vi "ShowErrorAndStatusAndStop.vi"(8 "error in":errorcluster, 10 "measured value in":dbl, 11 "measurement setting in":T1) -> ()   [LabVIEW 2011]
doc: "Shows errors and status of measurement."
uses:
  Measurement Setting.ctl
panel:
  out "measurement setting":T1
  out "measured value":dbl
  out "error":errorcluster
  # "Error occured! Run was terminated!"
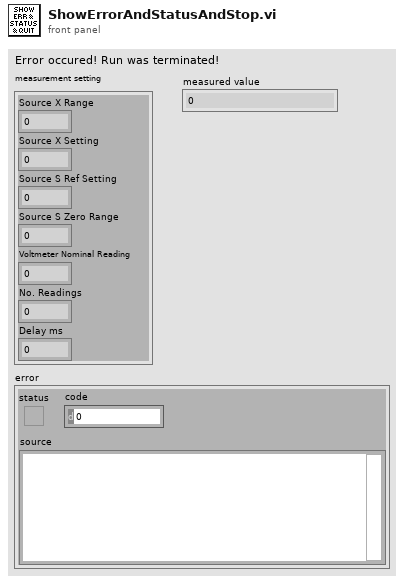
[diagram p1: front panel]
types:
  T1 = typedef "Measurement Setting.ctl" = cluster{"Source X Range":dbl, "Source X Setting":dbl, "Source S Ref Setting":dbl, "Source S Zero Range":dbl, "Voltmeter Nominal Reading":dbl, "No. Readings":dbl, "Delay ms":dbl}
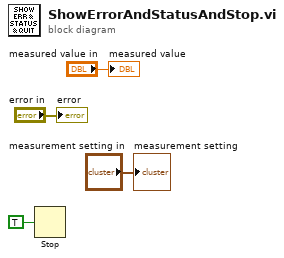
[diagram p0: block diagram]
diagram:
  n1 = Stop(stop? (T)=TRUE) -> ()
  "error" <- "error in"
  "measured value" <- "measured value in"
  "measurement setting" <- "measurement setting in"
